vi "HOST_856.vi"() -> ()   [LabVIEW 2018]
uses:
  <vilib>/userdefined/High Color/nirio_resource_hc.ctl
  <instrlib>/niDCPower/nidcpower.llb/niDCPower Measurement Type.ctl
  <vilib>/FPGAPlugInAG/PXI-7953R/niLvFpga_Open_PXI-7953R.vi
  <vilib>/rvi/interface/common/dynamic/niFpgaDynamicAddResources.vi
  <vilib>/FPGAPlugInAG/Dynamic/niLvFpga_Reset_Dynamic.vi
  <vilib>/FPGAPlugInAG/Dynamic/niLvFpga_Run_Dynamic.vi
  <vilib>/Utility/error.llb/Error Cluster From Error Code.vi
  <vilib>/rvi/errors/niLvFpgaAdjustHostInterfaceError.vi
  <vilib>/FPGAPlugInAG/Dynamic/niLvFpga_Close_Dynamic.vi
  <vilib>/rvi/interface/nirviOpenFPGA/nirviOpenFPGA.xnode
  FPGA Bitfiles/856_FPGATarget_TARGET856_CYBaMz25M7g.lvbitx
  <vilib>/rvi/interface/nirviMethod/nirviMethod.xnode
  <vilib>/rvi/interface/nirviReadWriteControl/nirviReadWriteControl.xnode
  <vilib>/rvi/interface/nirviCloseFPGA/nirviCloseFPGA.xnode
  NiFpgaLv.dll
  <vilib>/rvi/interface/Simulation/niFpgaSimulationCallBeginRW.vi
  <vilib>/FPGAPlugInAG/Dynamic/niLvFpga_ReadFifo_Dynamic.vi
  <vilib>/rvi/errors/niLvFpgaMergeErrorWithErrorCode.vi
panel:
  in  "Tab Control":enum32{"Рабочая", "Служебная"}(tab)
  out "Image":T1(plugin-control)
  in  "Frames":path=path "D:/VPL/LabView/DOZOR_856/DOZOR_856/FRAMES"
  out "Номер образца":string="0"
  in  "LOGS":path=path "D:/VPL/LabView/DOZOR_856/DOZOR_856/LOGS"
  in  "resource name":T2="PXI1Slot6"
  in  "1":refnum<k15>="PXI1Slot3" caption="instrument handle"
  in  "0":refnum<k15>="PXI1Slot2" caption="instrument handle"
  in  "2":refnum<k15>="PXI1Slot4" caption="instrument handle"
  in  "Стоп":bool
  in  "Питание":bool
  out "PS_LOW_cur":dbl caption="measurement" format="%_6g"
  in  "PS_LOW_curlim":dbl=0.1 caption="current limit" format="%_6p"
  in  "PS_LOW, V":dbl=-8.0 caption="voltage level" format="%_6p"
  in  "-15, V":dbl=-15.0 caption="voltage level" format="%_6p"
  out "-15_cur":dbl caption="measurement" format="%_6g"
  in  "-15_curlim":dbl=0.1 caption="current limit" format="%_6p"
  out "1V_cur":dbl caption="measurement" format="%_6g"
  in  "1V_curlim":dbl=0.1 caption="current limit" format="%_6p"
  in  "1V":dbl=1.0 caption="voltage level" format="%_6p"
  in  "2V":dbl=3.100000000000001 caption="voltage level" format="%_6p"
  in  "STAB, V":dbl=10.0 caption="voltage level" format="%_6p"
  out "DD_cur":dbl caption="measurement" format="%_6g"
  out "2V_cur":dbl caption="measurement" format="%_6g"
  out "PH_LOW_cur":dbl caption="measurement" format="%_6g"
  out "RD_cur":dbl caption="measurement" format="%_6g"
  out "STAB_cur":dbl caption="measurement" format="%_6g"
  out "ADC_cur":dbl caption="measurement" format="%_6g"
  in  "DD_curlim":dbl=0.2 caption="current limit" format="%_6p"
  in  "2V_curlim":dbl=0.1 caption="current limit" format="%_6p"
  in  "PH_LOW_curlim":dbl=0.2 caption="current limit" format="%_6p"
  in  "RD_curlim":dbl=0.1 caption="current limit" format="%_6p"
  in  "STAB_curlim":dbl=0.2 caption="current limit" format="%_6p"
  in  "ADC_curlim":dbl=0.2 caption="current limit" format="%_6p"
  in  "DD, V":dbl=18.900000000000013 caption="voltage level" format="%_6p"
  in  "PH_LOW, V":dbl=-4.000000000000002 caption="voltage level" format="%_6p"
  in  "RD, V":dbl=15.099999999999996 caption="voltage level" format="%_6p"
  in  "ADC, V":dbl=6.0 caption="voltage level" format="%_6p"
  in  "Линейки":bool
  out "СКО":dbl
  in  "LED":bool
  out "Configuration":bool[](array[boolean])
  out "АЦП прошит!":bool
  in  "2/4 V":enum16{"2V", "4V"}(ring)
  in  "3CH/1CH":enum16{"3CH", "1CH"}(ring)=enum."1CH"
  in  "Какой канал?":enum16{"OUT1", "OUT2", "OUT3"}(ring)
  in  "Прошить АЦП":bool
  in  "ПРИМЕЧАНИЕ":string
  in  "Какая фотка?":string
  in  "НЕПРЕРЫВНО":bool
  in  "文韧 世男!":bool
  out "Среднее":dbl
  out "FRAME_OK":bool
  in  "Запись Кадра":bool
  out "Канал":string="1"
  in  "ПЕРЕБОР?":bool
  out "ADC":i32
  out "1V":i32
  out "2V":i32
  out "STAB":i32
  out "RD":i32
  out "DD":i32
  out "-15":i32
  out "PH":i32
  out "PS":i32
  out "ADC":bool
  out "1V":bool
  out "2V":bool
  out "STAB":bool
  out "RD":bool
  out "DD":bool
  out "-15":bool
  out "PH":bool
  out "PS":bool
  in  "SIM_SEL":bool
  out "SEL":bool
  in  "ADC_selcur":dbl=0.15 caption="current limit" format="%_6p"
  in  "STAB_selcur":dbl=0.15 caption="current limit" format="%_6p"
  in  "-15_selcur":dbl=0.01 caption="current limit" format="%_6p"
  in  "1V_selcur":dbl=0.02 caption="current limit" format="%_6p"
  in  "RD_selcur":dbl=0.01 caption="current limit" format="%_6p"
  in  "2V_curlim":dbl=0.01 caption="current limit" format="%_6p"
  in  "DD_curlim":dbl=0.1 caption="current limit" format="%_6p"
  in  "PS_LOW_curlim":dbl=0.015 caption="current limit" format="%_6p"
  in  "PH_LOW_curlim":dbl=0.12 caption="current limit" format="%_6p"
  in  "ISO":dbl=1.0
  in  "+/- OUT2":enum16{"-", "+"}(ring)=enum."+"
  in  "Смещение, до 300_OUT2":dbl
  in  "+/- OUT3":enum16{"-", "+"}(ring)=enum."+"
  in  "Смещение, до 300_OUT3":dbl
  in  "+/- OUT1":enum16{"-", "+"}(ring)=enum."+"
  in  "Смещение, до 300_OUT1":dbl
  in  "Усиление (до 6)_OUT2":u8=1
  in  "Усиление (до 6)_OUT1":u8=1
  in  "Усиление (до 6)_OUT3":u8=1
  in  "Между кадрами, мс":u8=1
  in  "Усреднение":i32=1
  out "FRAME":u16[][](array[numeric])
  out "OUT":cluster{u16, u16, u16, u16}[][](array[cluster])
  in  "HIGH":u8=18
  in  "LOW":u8=7
  in  "HOR":u16=880
  in  "RG_2":u8=5
  in  "ADC_1":u8=5
  in  "ADC_2":u8=16
  in  "CDS2_1":u8=2
  in  "CDS2_2":u8=16
  in  "CDS1_1":u8=5
  in  "CDS1_2":u8=13
  in  "PS3_2":u16=1589
  in  "PS3_1":u16=934
  in  "PS1_1":u16=715
  in  "PS1_2":u16=1809
  in  "Сколько строк?":i32=110
  in  "2017":u16=2017
  in  "PS2_1":u16=496
  in  "PS2_2":u16=1151
  in  "PS4_1":u16=277
  in  "PS4_2":u16=1371
  in  "RG_1":u8=3
  in  "PH21_2":u8=13
  in  "PH21_1":u8=3
  in  "PH11_2":u8=13
  in  "PH11_1":u8=3
  in  "10":u8=20
  # "Для обычного кабеля"
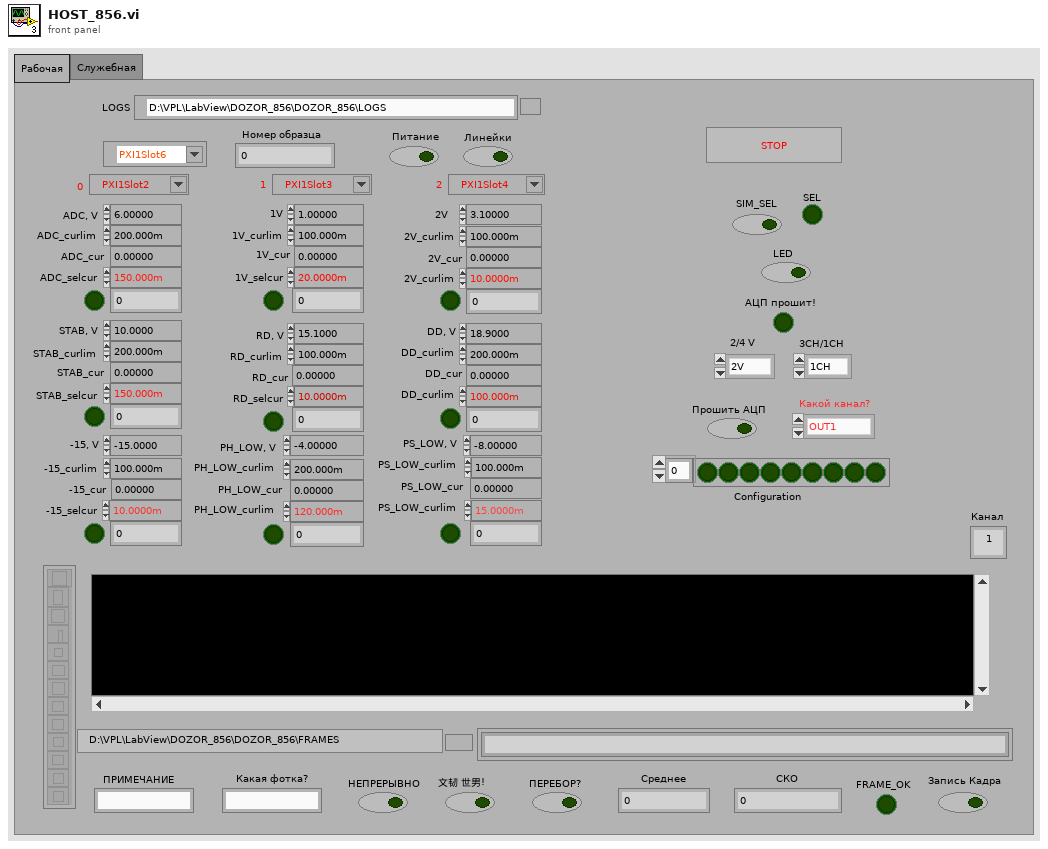
[diagram p1: front panel]
types:
  T1 = typedef "IMAQ Image.ctl" = refnum<image>
  T2 = typedef "nirio_resource_hc.ctl" = tag
  T3 = enum16{"open", "replace", "create", "open or create", "replace or create", "replace or create with confirmation"}
  T4 = typedef "niDCPower Measurement Type.ctl" = i32
  T5 = typedef "Image Type" = u32
  T6 = enum16{"Configuration", "MUX", "RED PGA", "GREEN PGA", "BLUE PGA", "RED OFF", "GREEN OFF", "BLUE OFF"}
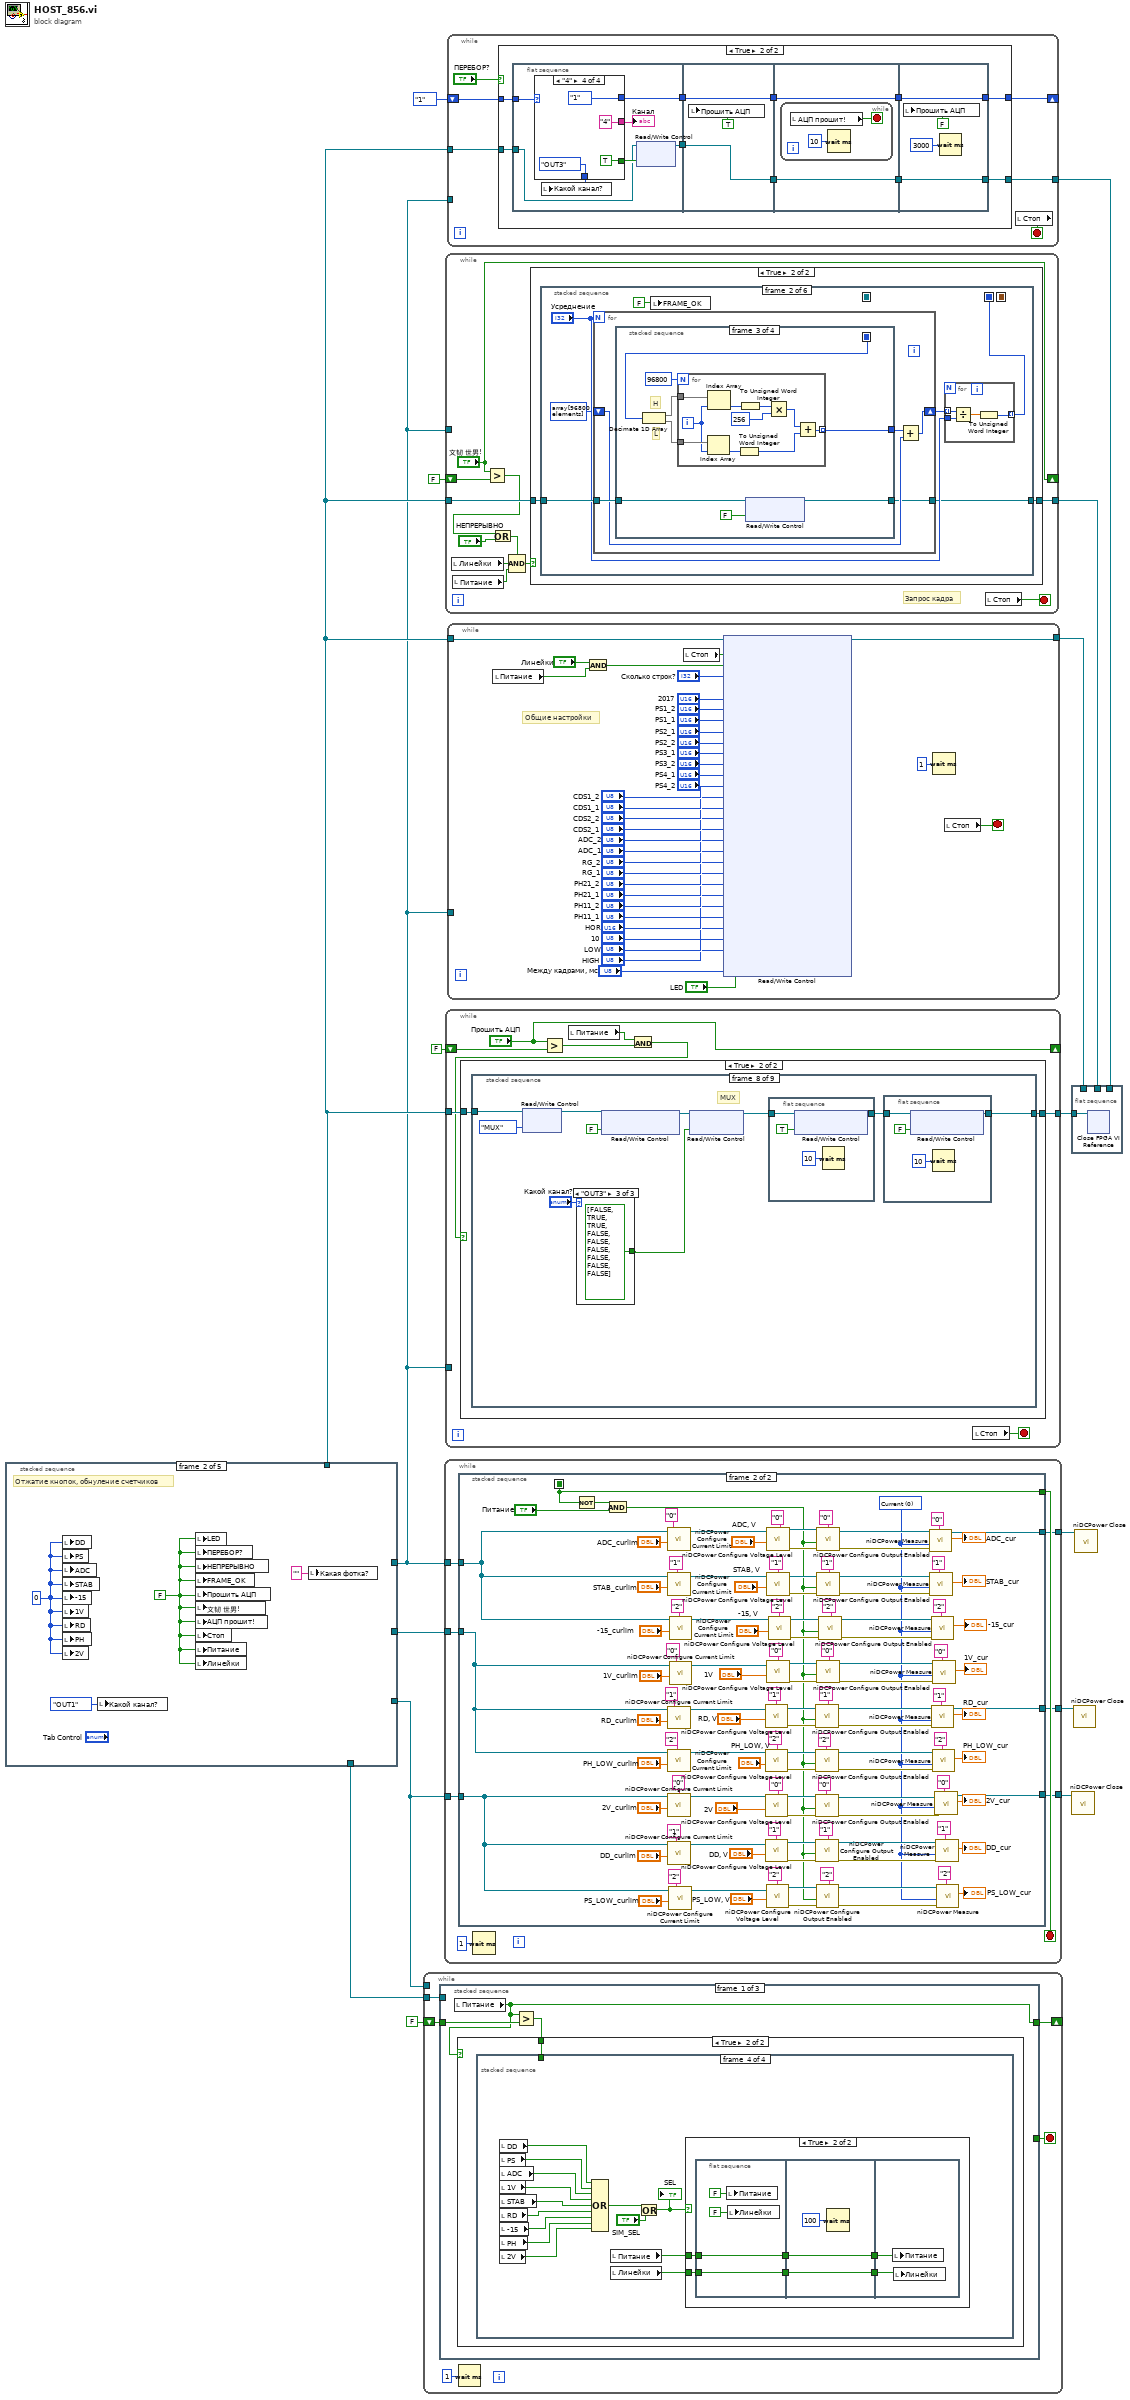
[diagram p0: block diagram]
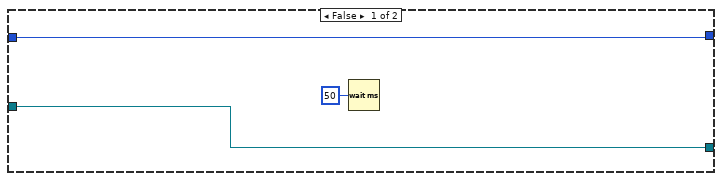
[diagram p2: hidden frame]
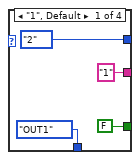
[diagram p3: hidden frame]
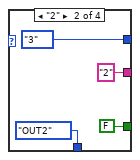
[diagram p4: hidden frame]
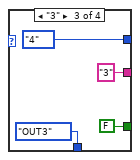
[diagram p5: hidden frame]
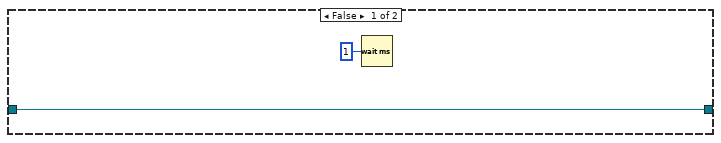
[diagram p6: hidden frame]
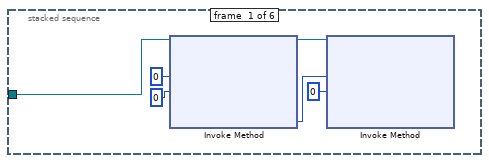
[diagram p7: hidden frame]
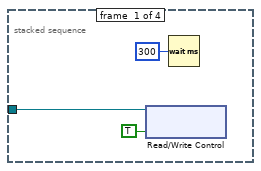
[diagram p8: hidden frame]
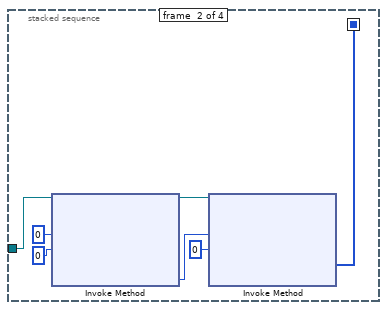
[diagram p9: hidden frame]
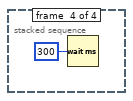
[diagram p10: hidden frame]
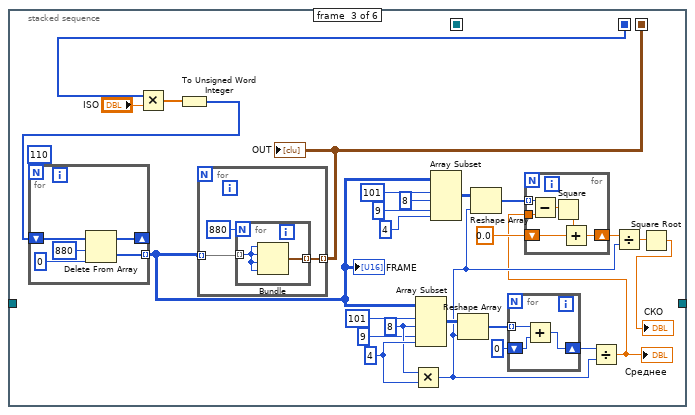
[diagram p11: hidden frame]
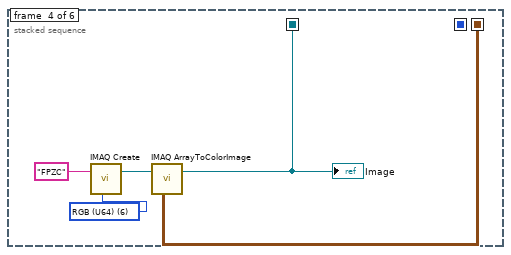
[diagram p12: hidden frame]
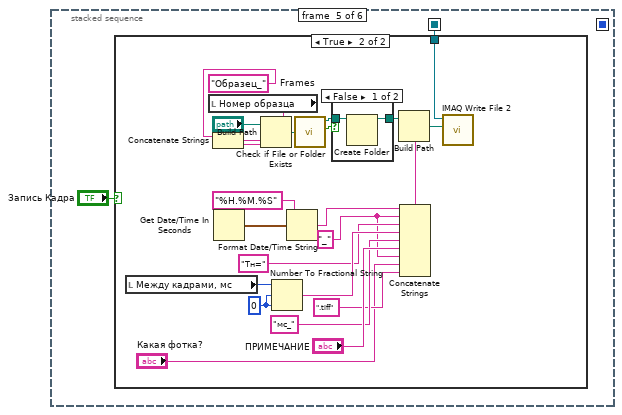
[diagram p13: hidden frame]
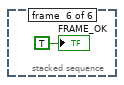
[diagram p16: hidden frame]
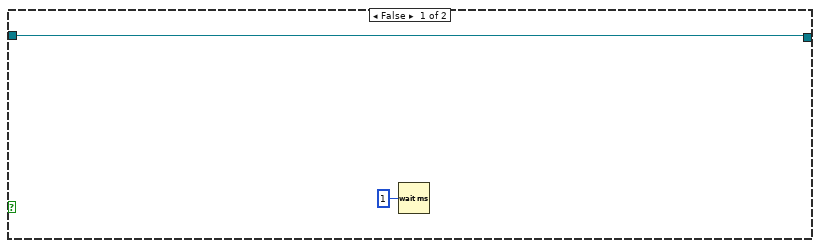
[diagram p17: hidden frame]
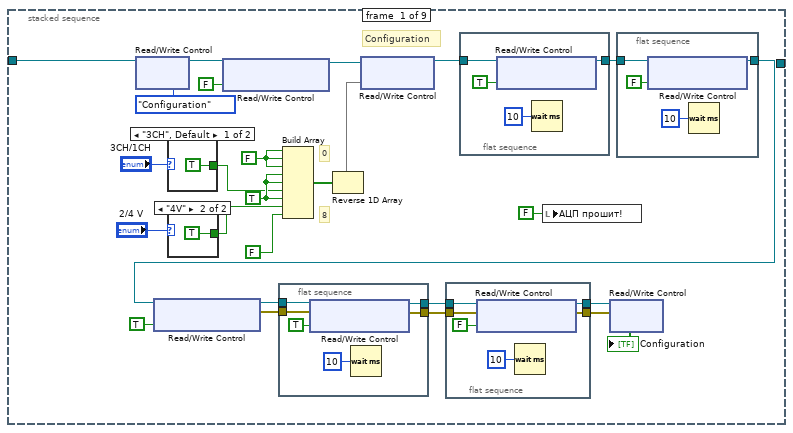
[diagram p18: hidden frame]
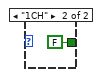
[diagram p19: hidden frame]
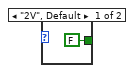
[diagram p20: hidden frame]
diagram:
  n1 = stacked-sequence {
    tunnel: [_ _ _ _ w67] -> w7
    tunnel: [_ _ _ _ w66] -> w5
    tunnel: [_ _ _ _ w65] -> w16
    tunnel: [_ _ _ w59 _] -> w9
    tunnel: [_ _ w22 _ _] -> w11
    frame #0 {
      n2 = call "Begin.vi"() -> ("Номер образца 2"=→"Номер образца":string)  [unwired: 11 in]
    }
    frame #1 {
      w18 = FALSE
      w19 = 0 ("DD")
      # "Отжатие кнопок, обнуление счетчиков"
      n3 = local write "DD"(w19) -> ()
      n4 = local write "PS"(w19) -> ()
      n5 = local write "ADC"(w19) -> ()
      n6 = local write "STAB"(w19) -> ()
      n7 = local write "-15"(w19) -> ()
      n8 = local write "1V"(w19) -> ()
      n9 = local write "RD"(w19) -> ()
      n10 = local write "PH"(w19) -> ()
      n11 = local write "2V"(w19) -> ()
      n12 = local write "Какой канал?"(enum16{"OUT1", "OUT2", "OUT3"}."OUT1" ("Какой канал?")) -> ()
      n13 = local write "LED"(w18) -> ()
      n14 = local write "ПЕРЕБОР?"(w18) -> ()
      n15 = local write "НЕПРЕРЫВНО"(w18) -> ()
      n16 = local write "FRAME_OK"(w18) -> ()
      n17 = local write "Прошить АЦП"(w18) -> ()
      n18 = local write "文韧 世男!"(w18) -> ()
      n19 = local write "АЦП прошит!"(w18) -> ()
      n20 = local write "Стоп"(w18) -> ()
      n21 = local write "Питание"(w18) -> ()
      n22 = local write "Линейки"(w18) -> ()
      n23 = local write "Какая фотка?"("" ("Какая фотка?")) -> ()
    }
    frame #2 {
      w24 = "\t"
      n24 = local read "Номер образца"() -> (w51:string)
      n25 = Build Path(base path="LOGS", name or relative path=w51) -> (appended path=w48:path)
      n26 = Get Date/Time In Seconds() -> (seconds since 1Jan1904=w45:timestamp)
      n27 = call <vilib>:"Check if File or Folder Exists.vi"("path"=w48) -> ("file or folder exists?"=w49:bool, "dup path"=w50:path)  [unwired: 8 in, 1 out]
      n28 = Format Date/Time String(time format string (%c)="%d %H.%M.%S", seconds (now)=w45) -> (date/time string=w43:string)  [unwired: 1 in]
      n29 = case shown="False" w49 {
        tunnel: w50 -> [w57 w58]
        tunnel: [w56 w58] -> w40
        frame False {
          n30 = Create Folder(path (use dialog)=w57) -> (created path=w56:path)  [unwired: 2 in, 2 out]
        }
        frame True {
        }
      }
      n31 = Concatenate Strings(w43, ".xls" ("string")) -> (w42:string)
      n32 = Build Path(base path=w40, name or relative path=w42) -> (appended path=w44:path)
      n33 = Open/Create/Replace File(file path (use dialog)=w44, operation (0:open)=T3."open or create", access (0:read/write)=enum16{"read/write", "read-only", "write-only"}."read/write") -> (refnum out=w46:refnum<file>)  [unwired: 3 in, 2 out]
      n34 = case shown="True" TRUE {
        tunnel: w46 -> [w52 w55]
        tunnel: [w52 w53] -> w41
        frame False {
        }
        frame True {
          n35 = Set File Position(refnum=w55, from (0:start)=enum16{"start", "end", "current"}."end") -> (refnum out=w53:refnum<file>)  [unwired: 2 in, 1 out]
        }
      }
      n36 = Format Into String(initial string=w41, "Time" ("input 1"), w24, "ADC_cur", w24, "STAB_cur", w24, "-15_cur", w24, "1_cur", w24, "RD_cur", w24, "PH_LOW_cur", w24, "2V_cur", w24, "DD_cur", w24, "PS_LOW_cur", "\r\n") -> (resulting string=w22:refnum<file>)  [unwired: 2 in, 1 out]
    }
    frame #3 {
      n37 = xnode "Open FPGA VI Reference"("resource name"="resource name") -> ("FPGA VI Reference Out"=w60:refnum<k20>, "error out"=w62:errorcluster)  [unwired: 1 in]
      n38 = xnode "Invoke Method"("FPGA VI Reference In"=w60, "error in"=w62) -> ("FPGA VI Reference Out"=w63:refnum<k20>, "error out"=w61:errorcluster)
      n39 = xnode "Invoke Method"("FPGA VI Reference In"=w63, "error in"=w61) -> ("FPGA VI Reference Out"=w59:refnum<k20>)  [unwired: 1 in, 1 out]
    }
    frame #4 {
      n40 = call <instrlib>:"niDCPower Initialize.vi"("resource name"="2") -> ("error out"=w73:errorcluster, "instrument handle out"=w70:refnum<k15>)  [unwired: 3 in, 6 out]
      n41 = call <instrlib>:"niDCPower Initialize.vi"("resource name"="1") -> ("error out"=w71:errorcluster, "instrument handle out"=w68:refnum<k15>)  [unwired: 3 in, 6 out]
      n42 = call <instrlib>:"niDCPower Initialize.vi"("resource name"="0") -> ("error out"=w72:errorcluster, "instrument handle out"=w69:refnum<k15>)  [unwired: 3 in, 6 out]
      n43 = call <instrlib>:"niDCPower Configure Voltage Level.vi"("error in (no error)"=w73, "voltage level"=0.0, "channel name"="0,1,2", "instrument handle"=w70) -> ("instrument handle out"=w67:refnum<k15>)  [unwired: 6 in, 1 out]
      n44 = call <instrlib>:"niDCPower Configure Voltage Level.vi"("error in (no error)"=w71, "voltage level"=0.0, "channel name"="0,1,2", "instrument handle"=w68) -> ("instrument handle out"=w65:refnum<k15>)  [unwired: 6 in, 1 out]
      n45 = call <instrlib>:"niDCPower Configure Voltage Level.vi"("error in (no error)"=w72, "voltage level"=0.0, "channel name"="0,1,2", "instrument handle"=w69) -> ("instrument handle out"=w66:refnum<k15>)  [unwired: 6 in, 1 out]
    }
  }
  n46 = while {
    shift-right: [w85] -> _
    shift-left: FALSE ("Питание") -> [w86]
    tunnel: w11 -> [w83]
    tunnel: w7 -> [_]
    stop <- w84 stop-if-true
    n47 = stacked-sequence {
      tunnel: [_ _ w228] -> w84
      tunnel: w86 -> [w90 _ _]
      tunnel: [w89 _ _] -> w85
      tunnel: w83 -> [_ w193 _]
      frame #0 {
        n48 = local read "Питание"() -> (w89:bool)
        n49 = Greater?(x=w89, y=w90) -> (0:w88:bool)
        n50 = case shown="True" w89 {
          tunnel: w88 -> [_ w91]
          frame False {
          }
          frame True {
            n51 = stacked-sequence {
              tunnel: w91 -> [w92 _ _ _]
              frame #0 {
                n52 = local read "SEL"() -> (w93:bool)
                n53 = Or(x=w92, y=w93) -> (x .or. y?=w94:bool)
                n54 = case shown="True" w94 {
                  frame False {
                  }
                  frame True {
                    n55 = flat-sequence {
                      frame #0 {
                        n56 = Wait (ms)(milliseconds to wait=u32 500) -> ()  [unwired: 1 out]
                      }
                      frame #1 {
                        n57 = local write "Прошить АЦП"(TRUE ("Прошить АЦП")) -> ()
                        n58 = Wait (ms)(milliseconds to wait=u32 100) -> ()  [unwired: 1 out]
                      }
                      frame #2 {
                        n59 = local write "Прошить АЦП"(FALSE ("Прошить АЦП")) -> ()
                      }
                    }
                  }
                }
              }
              frame #1 {
                n60 = local read "STAB_cur"() -> (w121:dbl)
                n61 = local read "1V_cur"() -> (w119:dbl)
                n62 = local read "2V_cur"() -> (w116:dbl)
                n63 = local read "ADC_cur"() -> (w124:dbl)
                n64 = Greater?(x=w119, y="1V_selcur") -> (0:→"1V":bool)
                n65 = Greater?(x=w116, y="2V_curlim") -> (0:→"2V":bool)
                n66 = Greater?(x=w121, y="STAB_selcur") -> (0:→"STAB":bool)
                n67 = Greater?(x=w124, y="ADC_selcur") -> (0:→"ADC":bool)
                n68 = local read "PH_LOW_cur"() -> (w104:dbl)
                n69 = local read "PS_LOW_cur"() -> (w113:dbl)
                n70 = local read "DD_cur"() -> (w110:dbl)
                n71 = local read "-15_cur"() -> (w101:dbl)
                n72 = local read "RD_cur"() -> (w107:dbl)
                n73 = Greater?(x=w107, y="RD_selcur") -> (0:→"RD":bool)
                n74 = Greater?(x=w104, y="PH_LOW_curlim") -> (0:→"PH":bool)
                n75 = Greater?(x=w101, y="-15_selcur") -> (0:→"-15":bool)
                n76 = Greater?(x=w110, y="DD_curlim") -> (0:→"DD":bool)
                n77 = Greater?(x=w113, y="PS_LOW_curlim") -> (0:→"PS":bool)
              }
              frame #2 {
                n78 = local read "ADC"() -> (w132:bool)
                n79 = local read "STAB"() -> (w131:bool)
                n80 = local read "-15"() -> (w130:bool)
                n81 = local read "1V"() -> (w129:bool)
                n82 = local read "DD"() -> (w134:bool)
                n83 = local read "PS"() -> (w133:bool)
                n84 = case shown="True" w134 {
                  frame False {
                  }
                  frame True {
                    n85 = local read "DD"() -> (w152:i32)
                    n86 = Increment(x=w152) -> (x+1=→"DD":i32)
                  }
                }
                n87 = case shown="True" w133 {
                  frame False {
                  }
                  frame True {
                    n88 = local read "PS"() -> (w150:i32)
                    n89 = Increment(x=w150) -> (x+1=→"PS":i32)
                  }
                }
                n90 = case shown="True" w132 {
                  frame False {
                  }
                  frame True {
                    n91 = local read "ADC"() -> (w148:i32)
                    n92 = Increment(x=w148) -> (x+1=→"ADC":i32)
                  }
                }
                n93 = case shown="True" w131 {
                  frame False {
                  }
                  frame True {
                    n94 = local read "STAB"() -> (w146:i32)
                    n95 = Increment(x=w146) -> (x+1=→"STAB":i32)
                  }
                }
                n96 = case shown="True" w130 {
                  frame False {
                  }
                  frame True {
                    n97 = local read "-15"() -> (w144:i32)
                    n98 = Increment(x=w144) -> (x+1=→"-15":i32)
                  }
                }
                n99 = case shown="True" w129 {
                  frame False {
                  }
                  frame True {
                    n100 = local read "1V"() -> (w142:i32)
                    n101 = Increment(x=w142) -> (x+1=→"1V":i32)
                  }
                }
                n102 = local read "RD"() -> (w128:bool)
                n103 = local read "2V"() -> (w126:bool)
                n104 = local read "PH"() -> (w127:bool)
                n105 = case shown="True" w127 {
                  frame False {
                  }
                  frame True {
                    n106 = local read "PH"() -> (w138:i32)
                    n107 = Increment(x=w138) -> (x+1=→"PH":i32)
                  }
                }
                n108 = case shown="True" w128 {
                  frame False {
                  }
                  frame True {
                    n109 = local read "RD"() -> (w140:i32)
                    n110 = Increment(x=w140) -> (x+1=→"RD":i32)
                  }
                }
                n111 = case shown="True" w126 {
                  frame False {
                  }
                  frame True {
                    n112 = local read "2V"() -> (w136:i32)
                    n113 = Increment(x=w136) -> (x+1=→"2V":i32)
                  }
                }
              }
              frame #3 {
                n114 = local read "DD"() -> (w165:bool)
                n115 = local read "PS"() -> (w164:bool)
                n116 = local read "ADC"() -> (w163:bool)
                n117 = local read "1V"() -> (w162:bool)
                n118 = local read "STAB"() -> (w161:bool)
                n119 = local read "RD"() -> (w160:bool)
                n120 = local read "-15"() -> (w159:bool)
                n121 = local read "PH"() -> (w158:bool)
                n122 = local read "2V"() -> (w157:bool)
                n123 = Compound Arithmetic op=OR(w165, w164, w163, w162, w161, w160, w159, w158, w157) -> (w156:bool)
                n124 = local read "Питание"() -> (w155:bool)
                n125 = local read "Линейки"() -> (w154:bool)
                n126 = Or(x=w156, y="SIM_SEL") -> (x .or. y?=w153:bool)
                "SEL" <- w153
                n127 = case shown="True" w153 {
                  tunnel: w155 -> [_ w173]
                  tunnel: w154 -> [_ w172]
                  frame False {
                    n128 = Wait (ms)(milliseconds to wait=u32 1) -> ()  [unwired: 1 out]
                  }
                  frame True {
                    n129 = flat-sequence {
                      tunnel: w173 -> [w177]
                      tunnel: w172 -> [w176]
                      tunnel: [w177] -> w170
                      tunnel: [w176] -> w168
                      tunnel: [w179] -> w171
                      tunnel: w170 -> [w179]
                      tunnel: [w178] -> w169
                      tunnel: w168 -> [w178]
                      tunnel: w171 -> [w182]
                      tunnel: w169 -> [w181]
                      frame #0 {
                        n130 = local write "Питание"(FALSE ("Питание")) -> ()
                        n131 = local write "Линейки"(FALSE ("Линейки")) -> ()
                      }
                      frame #1 {
                        n132 = Wait (ms)(milliseconds to wait=u32 100) -> ()  [unwired: 1 out]
                      }
                      frame #2 {
                        n133 = local write "Питание"(w182) -> ()
                        n134 = local write "Линейки"(w181) -> ()
                      }
                    }
                  }
                }
              }
            }
          }
        }
      }
      frame #1 {
        w203 = i16 0 ("width (-)")
        w206 = i16 3 ("width (-)")
        w204 = "\t"
        # "Логирование данных"
        n135 = local read "STAB"() -> (w201:i32)
        n136 = local read "ADC"() -> (w202:i32)
        n137 = local read "-15"() -> (w200:i32)
        n138 = local read "PH"() -> (w197:i32)
        n139 = local read "DD"() -> (w195:i32)
        n140 = local read "RD"() -> (w198:i32)
        n141 = local read "1V"() -> (w199:i32)
        n142 = local read "2V"() -> (w196:i32)
        n143 = local read "PS"() -> (w194:i32)
        n144 = Number To Fractional String(number=w202, width (-)=w203, precision (6)=w203) -> (F-format string=w191:string)  [unwired: 1 in]
        n145 = Number To Fractional String(number=w201, width (-)=w203, precision (6)=w203) -> (F-format string=w190:string)  [unwired: 1 in]
        n146 = Number To Fractional String(number=w200, width (-)=w203, precision (6)=w203) -> (F-format string=w189:string)  [unwired: 1 in]
        n147 = Number To Fractional String(number=w199, width (-)=w203, precision (6)=w203) -> (F-format string=w188:string)  [unwired: 1 in]
        n148 = Number To Fractional String(number=w198, width (-)=w203, precision (6)=w203) -> (F-format string=w187:string)  [unwired: 1 in]
        n149 = Number To Fractional String(number=w197, width (-)=w203, precision (6)=w203) -> (F-format string=w186:string)  [unwired: 1 in]
        n150 = Number To Fractional String(number=w196, width (-)=w203, precision (6)=w203) -> (F-format string=w185:string)  [unwired: 1 in]
        n151 = Number To Fractional String(number=w195, width (-)=w203, precision (6)=w203) -> (F-format string=w184:string)  [unwired: 1 in]
        n152 = Number To Fractional String(number=w194, width (-)=w203, precision (6)=w203) -> (F-format string=w183:string)  [unwired: 1 in]
        n153 = local read "PH_LOW_cur"() -> (w210:dbl)
        n154 = local read "PS_LOW_cur"() -> (w207:dbl)
        n155 = local read "STAB_cur"() -> (w214:dbl)
        n156 = local read "ADC_cur"() -> (w215:dbl)
        n157 = local read "DD_cur"() -> (w208:dbl)
        n158 = local read "-15_cur"() -> (w213:dbl)
        n159 = local read "RD_cur"() -> (w211:dbl)
        n160 = local read "1V_cur"() -> (w212:dbl)
        n161 = local read "2V_cur"() -> (w209:dbl)
        n162 = Number To Fractional String(number=w215, width (-)=w206, precision (6)=w206) -> (F-format string=w224:string)  [unwired: 1 in]
        n163 = Number To Fractional String(number=w214, width (-)=w206, precision (6)=w206) -> (F-format string=w223:string)  [unwired: 1 in]
        n164 = Number To Fractional String(number=w213, width (-)=w206, precision (6)=w206) -> (F-format string=w222:string)  [unwired: 1 in]
        n165 = Number To Fractional String(number=w212, width (-)=w206, precision (6)=w206) -> (F-format string=w221:string)  [unwired: 1 in]
        n166 = Number To Fractional String(number=w211, width (-)=w206, precision (6)=w206) -> (F-format string=w220:string)  [unwired: 1 in]
        n167 = Number To Fractional String(number=w210, width (-)=w206, precision (6)=w206) -> (F-format string=w219:string)  [unwired: 1 in]
        n168 = Number To Fractional String(number=w209, width (-)=w206, precision (6)=w206) -> (F-format string=w218:string)  [unwired: 1 in]
        n169 = Number To Fractional String(number=w208, width (-)=w206, precision (6)=w206) -> (F-format string=w217:string)  [unwired: 1 in]
        n170 = Number To Fractional String(number=w207, width (-)=w206, precision (6)=w206) -> (F-format string=w216:string)  [unwired: 1 in]
        n171 = Get Date/Time In Seconds() -> (seconds since 1Jan1904=w227:timestamp)
        n172 = Format Date/Time String(time format string (%c)="%d %H:%M:%S:%3u", seconds (now)=w227) -> (date/time string=w225:string)  [unwired: 1 in]
        n173 = Concatenate Strings(w225, w204, w224, w204, w223, w204, w222, w204, w221, w204, w220, w204, w219, w204, w218, w204, w217, w204, w216, w204, w191, w204, w190, w204, w189, w204, w188, w204, w187, w204, w186, w204, w185, w204, w184, w204, w183, "\r\n") -> (w226:string)
        n174 = Format Into String(initial string=w193, w226) -> ()  [unwired: 2 in, 2 out]
      }
      frame #2 {
        n175 = local read "Стоп"() -> (w228:bool)
      }
    }
    n176 = Wait (ms)(milliseconds to wait=u32 1) -> ()  [unwired: 1 out]
  }
  n177 = while {
    tunnel: w5 -> [w235]
    tunnel: w16 -> [w234]
    tunnel: w7 -> [w233]
    tunnel: [w231] -> w15
    tunnel: [w230] -> w14
    tunnel: [w229] -> w13
    stop <- w232 stop-if-true
    n178 = stacked-sequence {
      seq-local: ["Стоп" _] -> [_ w238]
      tunnel: w233 -> [_ w243]
      tunnel: [_ w284] -> w231
      tunnel: [_ w283] -> w230
      tunnel: [_ w282] -> w229
      tunnel: w235 -> [_ w242]
      tunnel: w234 -> [_ w241]
      tunnel: [_ w238] -> w232
      frame #0 {
      }
      frame #1 {
        w244 = T4 0 items=["Current", "Voltage"] ("measurement type")
        n179 = Not(x=w238) -> (.not. x?=w257:bool)
        n180 = And(x=w257, y="Питание") -> (x .and. y?=w239:bool)
        n181 = call <instrlib>:"niDCPower Configure Current Limit.vi"("current limit"="ADC_curlim", "channel name"="0", "instrument handle"=w242) -> ("instrument handle out"=w319:refnum<k15>)  [unwired: 7 in, 1 out]
        n182 = call <instrlib>:"niDCPower Configure Current Limit.vi"("current limit"="STAB_curlim", "channel name"="1", "instrument handle"=w242) -> ("instrument handle out"=w320:refnum<k15>)  [unwired: 7 in, 1 out]
        n183 = call <instrlib>:"niDCPower Configure Current Limit.vi"("current limit"="RD_curlim", "channel name"="1", "instrument handle"=w241) -> ("instrument handle out"=w321:refnum<k15>)  [unwired: 7 in, 1 out]
        n184 = call <instrlib>:"niDCPower Configure Current Limit.vi"("current limit"="PH_LOW_curlim", "channel name"="2", "instrument handle"=w241) -> ("instrument handle out"=w322:refnum<k15>)  [unwired: 7 in, 1 out]
        n185 = call <instrlib>:"niDCPower Configure Current Limit.vi"("current limit"="2V_curlim", "channel name"="0", "instrument handle"=w243) -> ("instrument handle out"=w323:refnum<k15>)  [unwired: 7 in, 1 out]
        n186 = call <instrlib>:"niDCPower Configure Current Limit.vi"("current limit"="DD_curlim", "channel name"="1", "instrument handle"=w243) -> ("instrument handle out"=w324:refnum<k15>)  [unwired: 7 in, 1 out]
        n187 = call <instrlib>:"niDCPower Configure Current Limit.vi"("current limit"="PS_LOW_curlim", "channel name"="2", "instrument handle"=w243) -> ("instrument handle out"=w250:refnum<k15>)  [unwired: 7 in, 1 out]
        n188 = call <instrlib>:"niDCPower Configure Current Limit.vi"("current limit"="-15_curlim", "channel name"="2", "instrument handle"=w242) -> ("instrument handle out"=w264:refnum<k15>)  [unwired: 7 in, 1 out]
        n189 = call <instrlib>:"niDCPower Configure Current Limit.vi"("current limit"="1V_curlim", "channel name"="0", "instrument handle"=w241) -> ("instrument handle out"=w275:refnum<k15>)  [unwired: 7 in, 1 out]
        n190 = call <instrlib>:"niDCPower Configure Voltage Level.vi"("voltage level"="RD, V", "channel name"="1", "instrument handle"=w321) -> ("error out"=w302:errorcluster, "instrument handle out"=w299:refnum<k15>)  [unwired: 7 in]
        n191 = call <instrlib>:"niDCPower Configure Voltage Level.vi"("voltage level"="PH_LOW, V", "channel name"="2", "instrument handle"=w322) -> ("error out"=w301:errorcluster, "instrument handle out"=w300:refnum<k15>)  [unwired: 7 in]
        n192 = call <instrlib>:"niDCPower Configure Voltage Level.vi"("voltage level"="2V", "channel name"="0", "instrument handle"=w323) -> ("error out"=w311:errorcluster, "instrument handle out"=w314:refnum<k15>)  [unwired: 7 in]
        n193 = call <instrlib>:"niDCPower Configure Voltage Level.vi"("voltage level"="DD, V", "channel name"="1", "instrument handle"=w324) -> ("error out"=w312:errorcluster, "instrument handle out"=w313:refnum<k15>)  [unwired: 7 in]
        n194 = call <instrlib>:"niDCPower Configure Voltage Level.vi"("voltage level"="PS_LOW, V", "channel name"="2", "instrument handle"=w250) -> ("error out"=w253:errorcluster, "instrument handle out"=w252:refnum<k15>)  [unwired: 7 in]
        n195 = call <instrlib>:"niDCPower Configure Voltage Level.vi"("voltage level"="ADC, V", "channel name"="0", "instrument handle"=w319) -> ("error out"=w289:errorcluster, "instrument handle out"=w292:refnum<k15>)  [unwired: 7 in]
        n196 = call <instrlib>:"niDCPower Configure Voltage Level.vi"("voltage level"="STAB, V", "channel name"="1", "instrument handle"=w320) -> ("error out"=w290:errorcluster, "instrument handle out"=w291:refnum<k15>)  [unwired: 7 in]
        n197 = call <instrlib>:"niDCPower Configure Voltage Level.vi"("voltage level"="1V", "channel name"="0", "instrument handle"=w275) -> ("error out"=w279:errorcluster, "instrument handle out"=w280:refnum<k15>)  [unwired: 7 in]
        n198 = call <instrlib>:"niDCPower Configure Voltage Level.vi"("voltage level"="-15, V", "channel name"="2", "instrument handle"=w264) -> ("error out"=w267:errorcluster, "instrument handle out"=w266:refnum<k15>)  [unwired: 7 in]
        n199 = call <instrlib>:"niDCPower Configure Output Enabled.vi"("error in (no error)"=w302, "output enabled"=w239, "channel name"="1", "instrument handle"=w299) -> ("error out"=w348:errorcluster, "instrument handle out"=w341:refnum<k15>)  [unwired: 6 in]
        n200 = call <instrlib>:"niDCPower Configure Output Enabled.vi"("error in (no error)"=w301, "output enabled"=w239, "channel name"="2", "instrument handle"=w300) -> ("error out"=w343:errorcluster, "instrument handle out"=w342:refnum<k15>)  [unwired: 6 in]
        n201 = call <instrlib>:"niDCPower Configure Output Enabled.vi"("error in (no error)"=w311, "output enabled"=w239, "channel name"="0", "instrument handle"=w314) -> ("error out"=w345:errorcluster, "instrument handle out"=w344:refnum<k15>)  [unwired: 6 in]
        n202 = call <instrlib>:"niDCPower Configure Output Enabled.vi"("error in (no error)"=w312, "output enabled"=w239, "channel name"="1", "instrument handle"=w313) -> ("error out"=w346:errorcluster, "instrument handle out"=w347:refnum<k15>)  [unwired: 6 in]
        n203 = call <instrlib>:"niDCPower Configure Output Enabled.vi"("error in (no error)"=w253, "output enabled"=w239, "channel name"="2", "instrument handle"=w252) -> ("error out"=w247:errorcluster, "instrument handle out"=w246:refnum<k15>)  [unwired: 6 in]
        n204 = call <instrlib>:"niDCPower Configure Output Enabled.vi"("error in (no error)"=w289, "output enabled"=w239, "channel name"="0", "instrument handle"=w292) -> ("error out"=w332:errorcluster, "instrument handle out"=w331:refnum<k15>)  [unwired: 6 in]
        n205 = call <instrlib>:"niDCPower Configure Output Enabled.vi"("error in (no error)"=w290, "output enabled"=w239, "channel name"="1", "instrument handle"=w291) -> ("error out"=w333:errorcluster, "instrument handle out"=w334:refnum<k15>)  [unwired: 6 in]
        n206 = call <instrlib>:"niDCPower Configure Output Enabled.vi"("error in (no error)"=w279, "output enabled"=w239, "channel name"="0", "instrument handle"=w280) -> ("error out"=w271:errorcluster, "instrument handle out"=w272:refnum<k15>)  [unwired: 6 in]
        n207 = call <instrlib>:"niDCPower Configure Output Enabled.vi"("error in (no error)"=w267, "output enabled"=w239, "channel name"="2", "instrument handle"=w266) -> ("error out"=w262:errorcluster, "instrument handle out"=w261:refnum<k15>)  [unwired: 6 in]
        n208 = call <instrlib>:"niDCPower Measure.vi"("error in (no error)"=w332, "measurement type"=w244, "channel name"="0", "instrument handle"=w331) -> ("measurement"=→"ADC_cur":dbl, "instrument handle out"=w284:refnum<k15>)  [unwired: 5 in, 1 out]
        n209 = call <instrlib>:"niDCPower Measure.vi"("error in (no error)"=w333, "measurement type"=w244, "channel name"="1", "instrument handle"=w334) -> ("measurement"=→"STAB_cur":dbl)  [unwired: 5 in, 2 out]
        n210 = call <instrlib>:"niDCPower Measure.vi"("error in (no error)"=w262, "measurement type"=w244, "channel name"="2", "instrument handle"=w261) -> ("measurement"=→"-15_cur":dbl)  [unwired: 5 in, 2 out]
        n211 = call <instrlib>:"niDCPower Measure.vi"("error in (no error)"=w348, "measurement type"=w244, "channel name"="1", "instrument handle"=w341) -> ("measurement"=→"RD_cur":dbl, "instrument handle out"=w283:refnum<k15>)  [unwired: 5 in, 1 out]
        n212 = call <instrlib>:"niDCPower Measure.vi"("error in (no error)"=w343, "measurement type"=w244, "channel name"="2", "instrument handle"=w342) -> ("measurement"=→"PH_LOW_cur":dbl)  [unwired: 5 in, 2 out]
        n213 = call <instrlib>:"niDCPower Measure.vi"("error in (no error)"=w271, "measurement type"=w244, "channel name"="0", "instrument handle"=w272) -> ("measurement"=→"1V_cur":dbl)  [unwired: 5 in, 2 out]
        n214 = call <instrlib>:"niDCPower Measure.vi"("error in (no error)"=w345, "measurement type"=w244, "channel name"="0", "instrument handle"=w344) -> ("measurement"=→"2V_cur":dbl, "instrument handle out"=w282:refnum<k15>)  [unwired: 5 in, 1 out]
        n215 = call <instrlib>:"niDCPower Measure.vi"("error in (no error)"=w346, "measurement type"=w244, "channel name"="1", "instrument handle"=w347) -> ("measurement"=→"DD_cur":dbl)  [unwired: 5 in, 2 out]
        n216 = call <instrlib>:"niDCPower Measure.vi"("error in (no error)"=w247, "measurement type"=w244, "channel name"="2", "instrument handle"=w246) -> ("measurement"=→"PS_LOW_cur":dbl)  [unwired: 5 in, 2 out]
      }
    }
    n217 = Wait (ms)(milliseconds to wait=u32 1) -> ()  [unwired: 1 out]
  }
  n218 = while {
    tunnel: w9 -> [w366]
    shift-right: ["文韧 世男!"] -> _
    shift-left: FALSE ("文韧 世男!") -> [w362]
    tunnel: [w357] -> w2
    tunnel: w5 -> [_]
    stop <- w367 stop-if-true
    # "Запрос кадра"
    n219 = local read "Линейки"() -> (w365:bool)
    n220 = local read "Питание"() -> (w364:bool)
    n221 = Greater?(x="文韧 世男!", y=w362) -> (0:w359:bool)
    n222 = Or(x=w359, y="НЕПРЕРЫВНО") -> (x .or. y?=w360:bool)
    n223 = Compound Arithmetic op=AND(w360, w365, w364) -> (w363:bool)
    n224 = case shown="True" w363 {
      tunnel: w366 -> [w368 w371]
      tunnel: [w368 w370] -> w357
      frame False {
        n225 = Wait (ms)(milliseconds to wait=u32 1) -> ()  [unwired: 1 out]
      }
      frame True {
        n226 = stacked-sequence {
          seq-local: [_ w383 _ _ _ _] -> [_ _ w438 _ _ _]
          seq-local: [_ _ w448 _ _ _] -> [_ _ _ w470 _ _]
          seq-local: [_ _ _ w469 _ _] -> [_ _ _ _ w474 _]
          tunnel: w371 -> [w372 w384 _ _ _ _]
          tunnel: [_ w378 _ _ _ _] -> w370
          frame #0 {
            n227 = xnode "Invoke Method"("FPGA VI Reference In"=w372, "Number of Elements"=u32 0, "Timeout (ms)"=0) -> ("FPGA VI Reference Out"=w377:refnum<k20>, "Elements Remaining"=w376:u32)  [unwired: 1 in, 2 out]
            n228 = xnode "Invoke Method"("FPGA VI Reference In"=w377, "Number of Elements"=w376, "Timeout (ms)"=0) -> ()  [unwired: 1 in, 4 out]
          }
          frame #1 {
            n229 = for {
              N: "Усреднение" -> [_]
              tunnel: w384 -> [w393]
              shift-right: [w390] -> w382
              shift-left: u64[] array[96800 elements] -> [w391]
              tunnel: [w389] -> w378
              n230 = stacked-sequence {
                seq-local: [_ w398 _ _] -> [_ _ w411 _]
                tunnel: w393 -> [w395 w397 w405 _]
                tunnel: [_ _ w407 _] -> w392
                tunnel: [_ _ w404 _] -> w389
                frame #0 {
                  n231 = xnode "Read/Write Control"("FPGA VI Reference In"=w395, "Кадр в FIFO"=TRUE) -> ()  [unwired: 1 in, 2 out]
                  n232 = Wait (ms)(milliseconds to wait=u32 300) -> ()  [unwired: 1 out]
                }
                frame #1 {
                  n233 = xnode "Invoke Method"("FPGA VI Reference In"=w397, "Number of Elements"=u32 0, "Timeout (ms)"=0) -> ("FPGA VI Reference Out"=w400:refnum<k20>, "Elements Remaining"=w399:u32)  [unwired: 1 in, 2 out]
                  n234 = xnode "Invoke Method"("FPGA VI Reference In"=w400, "Number of Elements"=w399, "Timeout (ms)"=0) -> ("Data"=w398:u8[])  [unwired: 1 in, 3 out]
                }
                frame #2 {
                  # "L"
                  # "H"
                  n235 = Decimate 1D Array(w411) -> (w410:u8[], w409:u8[])
                  n236 = for {
                    N: 96800 -> [_]
                    tunnel: w410 -> [w421]
                    tunnel: w409 -> [w420]
                    tunnel: [w412] -> w407 mode=indexing
                    i -> [w419]
                    n237 = Index Array(array=w420, index=w419) -> (element=w417:u8)
                    n238 = Index Array(array=w421, index=w419) -> (element=w418:u8)
                    n239 = To Unsigned Word Integer(number=w417) -> (unsigned 16bit integer=w413:u16)
                    n240 = To Unsigned Word Integer(number=w418) -> (unsigned 16bit integer=w416:u16)
                    n241 = Multiply(x=w416, y=u16 256) -> (x*y=w414:u16)
                    n242 = Add(x=w414, y=w413) -> (x+y=w412:u16)
                  }
                  n243 = xnode "Read/Write Control"("FPGA VI Reference In"=w405, "Кадр в FIFO"=FALSE) -> ("FPGA VI Reference Out"=w404:refnum<k20>)  [unwired: 1 in, 1 out]
                }
                frame #3 {
                  n244 = Wait (ms)(milliseconds to wait=u32 300) -> ()  [unwired: 1 out]
                }
              }
              n245 = Add(x=w392, y=w391) -> (x+y=w390:u64[])
            }
            n246 = local write "FRAME_OK"(FALSE ("FRAME_OK")) -> ()
            n247 = for {
              tunnel: w382 -> [w388] mode=indexing
              tunnel: "Усреднение" -> [w387]
              tunnel: [w385] -> w383 mode=indexing
              n248 = Divide(x=w388, y=w387) -> (x/y=w386:dbl)
              n249 = To Unsigned Word Integer(number=w386) -> (unsigned 16bit integer=w385:u16)
            }
          }
          frame #2 {
            w443 = 4 ("length")
            w442 = 8 ("length")
            n250 = Multiply(x=w438, y="ISO") -> (x*y=w437:dbl[])
            n251 = To Unsigned Word Integer(number=w437) -> (unsigned 16bit integer=w436:u16[])
            n252 = for {
              N: 110 -> [_]
              tunnel: [w465] -> w423 mode=indexing
              shift-right: [w464] -> _
              shift-left: w436 -> [w468]
              n253 = Delete From Array(array=w468, length=880, index=0) -> (deleted portion=w465:u16[], array with subset deleted=w464:u16[])
            }
            "FRAME" <- w423
            n254 = for {
              tunnel: w423 -> [w460] mode=indexing
              tunnel: [w459] -> w448 mode=indexing
              n255 = for {
                N: 880 -> [_]
                tunnel: [w463] -> w459 mode=indexing
                tunnel: w460 -> [w462] mode=indexing
                n256 = Bundle(w462, w462, w462, w462) -> (w463:cluster{u16, u16, u16, u16})  [unwired: 1 in]
              }
            }
            "OUT" <- w448
            n257 = Multiply(x=w442, y=w443) -> (x*y=w427:i32)
            n258 = Array Subset(array=w423, index (row)=101 ("index"), length (row)=w442, index (col)=9 ("index"), length (col)=w443) -> (w445:u16[][])
            n259 = Array Subset(array=w423, index (row)=101 ("index"), length (row)=8 ("length"), index (col)=9 ("index"), length (col)=4 ("length")) -> (w434:u16[][])
            n260 = Reshape Array(w445, w427) -> (w446:u16[])
            n261 = Reshape Array(w434, w427) -> (w430:u16[])
            n262 = for {
              tunnel: w446 -> [w458] mode=indexing
              shift-right: [w456] -> w447
              shift-left: u64 0 -> [w457]
              n263 = Add(x=w458, y=w457) -> (x+y=w456:u64)
            }
            n264 = Divide(x=w447, y=w427) -> (x/y=w424:dbl)
            "Среднее" <- w424
            n265 = for {
              tunnel: w424 -> [w454]
              tunnel: w430 -> [w455] mode=indexing
              shift-right: [w450] -> w435
              shift-left: 0.0 -> [w452]
              n266 = Subtract(x=w455, y=w454) -> (x-y=w453:dbl)
              n267 = Square(x=w453) -> (x^2=w451:dbl)
              n268 = Add(x=w451, y=w452) -> (x+y=w450:dbl)
            }
            n269 = Divide(x=w435, y=w427) -> (x/y=w426:dbl)
            n270 = Square Root(x=w426) -> (sqrt(x)=→"СКО":dbl)
          }
          frame #3 {
            w471 = T5 6 items=["Grayscale (U8)", "Grayscale (I16)", "Grayscale (SGL)", "Complex (CSG)", "RGB (U32)", "HSL (U32)", "RGB (U64)"] ("Image Type")
            n271 = call "IMAQ Create"("Image Name"="FPZC", "Image Type"=w471) -> ("New Image"=w473:T1)  [unwired: 3 in, 1 out]
            n272 = call "IMAQ ArrayToColorImage"("Image"=w473, "Image Pixels (U64)"=w470) -> ("Image Out"=w469:T1)  [unwired: 3 in, 1 out]
            "Image" <- w469
          }
          frame #4 {
            n273 = case shown="True" "Запись Кадра" {
              tunnel: w474 -> [_ w479]
              frame False {
              }
              frame True {
                w484 = i16 0 ("precision (6)")
                w478 = "_"
                n274 = local read "Между кадрами, мс"() -> (w496:u8)
                n275 = local read "Номер образца"() -> (w490:string)
                n276 = Concatenate Strings("Образец_" ("string"), w490) -> (w485:string)
                n277 = Get Date/Time In Seconds() -> (seconds since 1Jan1904=w493:timestamp)
                n278 = Build Path(base path="Frames", name or relative path=w485) -> (appended path=w489:path)
                n279 = Number To Fractional String(number=w496, width (-)=w484, precision (6)=w484) -> (F-format string=w497:string)  [unwired: 1 in]
                n280 = Format Date/Time String(time format string (%c)="%H.%M.%S", seconds (now)=w493) -> (date/time string=w495:string)  [unwired: 1 in]
                n281 = call <vilib>:"Check if File or Folder Exists.vi"("path"=w489) -> ("file or folder exists?"=w488:bool, "dup path"=w487:path)  [unwired: 8 in, 1 out]
                n282 = case shown="False" w488 {
                  tunnel: w487 -> [w500 w501]
                  tunnel: [w499 w501] -> w494
                  frame False {
                    n283 = Create Folder(path (use dialog)=w500) -> (created path=w499:path)  [unwired: 2 in, 2 out]
                  }
                  frame True {
                  }
                }
                n284 = Concatenate Strings(w495, w478, "Тн=" ("string"), w497, "мс_" ("string"), "ПРИМЕЧАНИЕ", w478, "Какая фотка?", ".tiff" ("element")) -> (w491:string)
                n285 = Build Path(base path=w494, name or relative path=w491) -> (appended path=w492:path)
                n286 = call-poly "IMAQ Write File 2"("File Path"=w492, "Image"=w479) -> ()  [unwired: 8 in, 2 out]
              }
            }
          }
          frame #5 {
            "FRAME_OK" <- TRUE
          }
        }
      }
    }
    n287 = local read "Стоп"() -> (w367:bool)
  }
  n288 = while {
    tunnel: w9 -> [w509]
    shift-right: ["Прошить АЦП"] -> _
    shift-left: FALSE -> [w508]
    tunnel: [w503] -> w4
    tunnel: w5 -> [_]
    stop <- w510 stop-if-true
    n289 = Greater?(x="Прошить АЦП", y=w508) -> (0:w506:bool)
    n290 = local read "Питание"() -> (w504:bool)
    n291 = And(x=w504, y=w506) -> (x .and. y?=w505:bool)
    n292 = case shown="True" w505 {
      tunnel: w509 -> [w511 w514]
      tunnel: [w511 w513] -> w503
      frame False {
        n293 = Wait (ms)(milliseconds to wait=u32 1) -> ()  [unwired: 1 out]
      }
      frame True {
        n294 = stacked-sequence {
          tunnel: w514 -> [w540 w580 w594 w623 w667 w677 w702 w736 _]
          tunnel: [_ _ _ _ _ _ _ w727 _] -> w513
          frame #0 {
            w536 = TRUE ("element")
            w537 = FALSE
            # "8"
            # "0"
            # "Configuration"
            n295 = xnode "Read/Write Control"("FPGA VI Reference In"=w540, "Enum"=T6."Configuration") -> ("FPGA VI Reference Out"=w527:refnum<k20>)  [unwired: 1 in, 1 out]
            n296 = xnode "Read/Write Control"("FPGA VI Reference In"=w517, "Read(T)/Write(F)"=TRUE) -> ("FPGA VI Reference Out"=w523:refnum<k20>, "error out"=w522:errorcluster)  [unwired: 1 in]
            n297 = case shown="\"3CH\", Default" "3CH/1CH" {
              tunnel: [TRUE FALSE] -> w535
              frame "3CH", Default {
              }
              frame "1CH" {
              }
            }
            n298 = case shown="\"4V\"" "2/4 V" {
              tunnel: [FALSE TRUE] -> w533
              frame "2V", Default {
              }
              frame "4V" {
              }
            }
            n299 = xnode "Read/Write Control"("FPGA VI Reference In"=w527, "Read(T)/Write(F)"=FALSE) -> ("FPGA VI Reference Out"=w525:refnum<k20>)  [unwired: 1 in, 1 out]
            n300 = flat-sequence {
              tunnel: w523 -> [w552]
              tunnel: w522 -> [w551]
              tunnel: [w550] -> w521
              tunnel: [w549] -> w520
              frame #0 {
                n301 = xnode "Read/Write Control"("FPGA VI Reference In"=w552, "error in"=w551, "Конфигурация"=TRUE) -> ("FPGA VI Reference Out"=w550:refnum<k20>, "error out"=w549:errorcluster)
                n302 = Wait (ms)(milliseconds to wait=u32 10) -> ()  [unwired: 1 out]
              }
            }
            n303 = Build Array(w537, w537, w537, w536, w536, w535, w536, w533, FALSE) -> (w538:bool[])
            n304 = Reverse 1D Array(array=w538) -> (reversed array=w530:bool[])
            n305 = xnode "Read/Write Control"("FPGA VI Reference In"=w525, "Write Data"=w530) -> ("FPGA VI Reference Out"=w529:refnum<k20>)  [unwired: 1 in, 1 out]
            n306 = flat-sequence {
              tunnel: w521 -> [w546]
              tunnel: w520 -> [w545]
              tunnel: [w543] -> w519
              tunnel: [w542] -> w518
              frame #0 {
                n307 = xnode "Read/Write Control"("FPGA VI Reference In"=w546, "error in"=w545, "Конфигурация"=FALSE) -> ("FPGA VI Reference Out"=w543:refnum<k20>, "error out"=w542:errorcluster)
                n308 = Wait (ms)(milliseconds to wait=u32 10) -> ()  [unwired: 1 out]
              }
            }
            n309 = flat-sequence {
              tunnel: w529 -> [w560]
              tunnel: [w558] -> w528
              frame #0 {
                n310 = xnode "Read/Write Control"("FPGA VI Reference In"=w560, "Конфигурация"=TRUE) -> ("FPGA VI Reference Out"=w558:refnum<k20>)  [unwired: 1 in, 1 out]
                n311 = Wait (ms)(milliseconds to wait=u32 10) -> ()  [unwired: 1 out]
              }
            }
            n312 = local write "АЦП прошит!"(FALSE ("АЦП прошит!")) -> ()
            n313 = xnode "Read/Write Control"("FPGA VI Reference In"=w519, "error in"=w518) -> ("READ"=→"Configuration":bool[])  [unwired: 2 out]
            n314 = flat-sequence {
              tunnel: w528 -> [w556]
              tunnel: [w554] -> w517
              frame #0 {
                n315 = xnode "Read/Write Control"("FPGA VI Reference In"=w556, "Конфигурация"=FALSE) -> ("FPGA VI Reference Out"=w554:refnum<k20>)  [unwired: 1 in, 1 out]
                n316 = Wait (ms)(milliseconds to wait=u32 10) -> ()  [unwired: 1 out]
              }
            }
          }
          frame #1 {
            # "GREEN_OFFSET"
            n317 = case shown="\"-\", Default" "+/- OUT2" {
              tunnel: [TRUE FALSE] -> w567
              frame "-", Default {
              }
              frame "+" {
              }
            }
            n318 = Quotient & Remainder(x="Смещение, до 300_OUT2", y=1.171875) -> (floor(x/y)=w572:dbl)  [unwired: 1 out]
            n319 = xnode "Read/Write Control"("FPGA VI Reference In"=w580, "Enum"=T6."GREEN OFF" ("OFFSET")) -> ("FPGA VI Reference Out"=w579:refnum<k20>, "error out"=w578:errorcluster)  [unwired: 1 in]
            n320 = Subtract(x=w572, y=1.0) -> (x-y=w569:dbl)
            n321 = To Unsigned Byte Integer(number=w569) -> (unsigned 8bit integer=w568:u8)
            n322 = xnode "Read/Write Control"("FPGA VI Reference In"=w579, "error in"=w578, "Read(T)/Write(F)"=FALSE) -> ("FPGA VI Reference Out"=w577:refnum<k20>)  [unwired: 1 out]
            n323 = Number To Boolean Array(number=w568) -> (Boolean array=w566:bool[])
            n324 = Reverse 1D Array(array=w566) -> (reversed array=w565:bool[])
            n325 = Build Array (concatenate)(w567, w565) -> (w570:bool[])
            n326 = xnode "Read/Write Control"("FPGA VI Reference In"=w577, "Write Data"=w570) -> ("FPGA VI Reference Out"=w582:refnum<k20>)  [unwired: 1 in, 1 out]
            n327 = flat-sequence {
              tunnel: w582 -> [w593]
              tunnel: [w591] -> w581
              frame #0 {
                n328 = xnode "Read/Write Control"("FPGA VI Reference In"=w593, "Конфигурация"=TRUE) -> ("FPGA VI Reference Out"=w591:refnum<k20>)  [unwired: 1 in, 1 out]
                n329 = Wait (ms)(milliseconds to wait=u32 10) -> ()  [unwired: 1 out]
              }
            }
            n330 = flat-sequence {
              tunnel: w581 -> [w589]
              tunnel: [w587] -> _
              frame #0 {
                n331 = xnode "Read/Write Control"("FPGA VI Reference In"=w589, "Конфигурация"=FALSE) -> ("FPGA VI Reference Out"=w587:refnum<k20>)  [unwired: 1 in, 1 out]
                n332 = Wait (ms)(milliseconds to wait=u32 10) -> ()  [unwired: 1 out]
              }
            }
          }
          frame #2 {
            # "RED_OFFSET"
            n333 = case shown="\"-\", Default" "+/- OUT3" {
              tunnel: [TRUE FALSE] -> w610
              frame "-", Default {
              }
              frame "+" {
              }
            }
            n334 = Quotient & Remainder(x="Смещение, до 300_OUT3", y=1.171875) -> (floor(x/y)=w605:dbl)  [unwired: 1 out]
            n335 = xnode "Read/Write Control"("FPGA VI Reference In"=w594, "Enum"=T6."RED OFF" ("OFFSET")) -> ("FPGA VI Reference Out"=w601:refnum<k20>, "error out"=w602:errorcluster)  [unwired: 1 in]
            n336 = Subtract(x=w605, y=1.0) -> (x-y=w608:dbl)
            n337 = To Unsigned Byte Integer(number=w608) -> (unsigned 8bit integer=w609:u8)
            n338 = xnode "Read/Write Control"("FPGA VI Reference In"=w601, "error in"=w602, "Read(T)/Write(F)"=FALSE) -> ("FPGA VI Reference Out"=w603:refnum<k20>)  [unwired: 1 out]
            n339 = Number To Boolean Array(number=w609) -> (Boolean array=w611:bool[])
            n340 = Reverse 1D Array(array=w611) -> (reversed array=w612:bool[])
            n341 = Build Array (concatenate)(w610, w612) -> (w607:bool[])
            n342 = xnode "Read/Write Control"("FPGA VI Reference In"=w603, "Write Data"=w607) -> ("FPGA VI Reference Out"=w599:refnum<k20>)  [unwired: 1 in, 1 out]
            n343 = flat-sequence {
              tunnel: w599 -> [w622]
              tunnel: [w620] -> w600
              frame #0 {
                n344 = xnode "Read/Write Control"("FPGA VI Reference In"=w622, "Конфигурация"=TRUE) -> ("FPGA VI Reference Out"=w620:refnum<k20>)  [unwired: 1 in, 1 out]
                n345 = Wait (ms)(milliseconds to wait=u32 10) -> ()  [unwired: 1 out]
              }
            }
            n346 = flat-sequence {
              tunnel: w600 -> [w618]
              tunnel: [w616] -> _
              frame #0 {
                n347 = xnode "Read/Write Control"("FPGA VI Reference In"=w618, "Конфигурация"=FALSE) -> ("FPGA VI Reference Out"=w616:refnum<k20>)  [unwired: 1 in, 1 out]
                n348 = Wait (ms)(milliseconds to wait=u32 10) -> ()  [unwired: 1 out]
              }
            }
          }
          frame #3 {
            # "BLUE_OFFSET"
            n349 = case shown="\"-\", Default" "+/- OUT1" {
              tunnel: [TRUE FALSE] -> w639
              frame "-", Default {
              }
              frame "+" {
              }
            }
            n350 = Quotient & Remainder(x="Смещение, до 300_OUT1", y=1.171875) -> (floor(x/y)=w634:dbl)  [unwired: 1 out]
            n351 = xnode "Read/Write Control"("FPGA VI Reference In"=w623, "Enum"=T6."BLUE OFF" ("OFFSET")) -> ("FPGA VI Reference Out"=w630:refnum<k20>, "error out"=w631:errorcluster)  [unwired: 1 in]
            n352 = Subtract(x=w634, y=1.0) -> (x-y=w637:dbl)
            n353 = To Unsigned Byte Integer(number=w637) -> (unsigned 8bit integer=w638:u8)
            n354 = xnode "Read/Write Control"("FPGA VI Reference In"=w630, "error in"=w631, "Read(T)/Write(F)"=FALSE) -> ("FPGA VI Reference Out"=w632:refnum<k20>)  [unwired: 1 out]
            n355 = Number To Boolean Array(number=w638) -> (Boolean array=w640:bool[])
            n356 = Reverse 1D Array(array=w640) -> (reversed array=w641:bool[])
            n357 = Build Array (concatenate)(w639, w641) -> (w636:bool[])
            n358 = xnode "Read/Write Control"("FPGA VI Reference In"=w632, "Write Data"=w636) -> ("FPGA VI Reference Out"=w628:refnum<k20>)  [unwired: 1 in, 1 out]
            n359 = flat-sequence {
              tunnel: w628 -> [w651]
              tunnel: [w649] -> w629
              frame #0 {
                n360 = xnode "Read/Write Control"("FPGA VI Reference In"=w651, "Конфигурация"=TRUE) -> ("FPGA VI Reference Out"=w649:refnum<k20>)  [unwired: 1 in, 1 out]
                n361 = Wait (ms)(milliseconds to wait=u32 10) -> ()  [unwired: 1 out]
              }
            }
            n362 = flat-sequence {
              tunnel: w629 -> [w647]
              tunnel: [w645] -> _
              frame #0 {
                n363 = xnode "Read/Write Control"("FPGA VI Reference In"=w647, "Конфигурация"=FALSE) -> ("FPGA VI Reference Out"=w645:refnum<k20>)  [unwired: 1 in, 1 out]
                n364 = Wait (ms)(milliseconds to wait=u32 10) -> ()  [unwired: 1 out]
              }
            }
          }
          frame #4 {
            w662 = FALSE
            # "GREEN PGA"
            n365 = Decrement(x="Усиление (до 6)_OUT2") -> (x-1=w654:u8)
            n366 = Multiply(x=w654, y=378) -> (x*y=w656:i32)
            n367 = Multiply(x="Усиление (до 6)_OUT2", y=5) -> (x*y=w659:i32)
            n368 = xnode "Read/Write Control"("FPGA VI Reference In"=w667, "Enum"=T6."GREEN PGA" ("PGA")) -> ("FPGA VI Reference Out"=w665:refnum<k20>)  [unwired: 1 in, 1 out]
            n369 = Divide(x=w656, y=w659) -> (x/y=w660:dbl)
            n370 = Number To Boolean Array(number=w660) -> (Boolean array=w653:bool[])
            n371 = xnode "Read/Write Control"("FPGA VI Reference In"=w665, "Read(T)/Write(F)"=FALSE) -> ("FPGA VI Reference Out"=w664:refnum<k20>)  [unwired: 1 in, 1 out]
            n372 = Build Array (concatenate)(w662, w662, w662, w653) -> (w661:bool[])
            n373 = xnode "Read/Write Control"("FPGA VI Reference In"=w664, "Write Data"=w661) -> ("FPGA VI Reference Out"=w666:refnum<k20>)  [unwired: 1 in, 1 out]
            n374 = flat-sequence {
              tunnel: [w675] -> w668
              tunnel: w666 -> [w674]
              frame #0 {
                n375 = xnode "Read/Write Control"("FPGA VI Reference In"=w674, "Конфигурация"=TRUE) -> ("FPGA VI Reference Out"=w675:refnum<k20>)  [unwired: 1 in, 1 out]
                n376 = Wait (ms)(milliseconds to wait=u32 10) -> ()  [unwired: 1 out]
              }
            }
            n377 = flat-sequence {
              tunnel: w668 -> [w672]
              tunnel: [w670] -> _
              frame #0 {
                n378 = xnode "Read/Write Control"("FPGA VI Reference In"=w672, "Конфигурация"=FALSE) -> ("FPGA VI Reference Out"=w670:refnum<k20>)  [unwired: 1 in, 1 out]
                n379 = Wait (ms)(milliseconds to wait=u32 10) -> ()  [unwired: 1 out]
              }
            }
          }
          frame #5 {
            w680 = FALSE
            # "BLUE PGA"
            n380 = Decrement(x="Усиление (до 6)_OUT1") -> (x-1=w684:u8)
            n381 = Multiply(x=w684, y=378) -> (x*y=w685:i32)
            n382 = Multiply(x="Усиление (до 6)_OUT1", y=5) -> (x*y=w687:i32)
            n383 = xnode "Read/Write Control"("FPGA VI Reference In"=w677, "Enum"=T6."BLUE PGA" ("PGA")) -> ("FPGA VI Reference Out"=w691:refnum<k20>)  [unwired: 1 in, 1 out]
            n384 = Divide(x=w685, y=w687) -> (x/y=w688:dbl)
            n385 = Number To Boolean Array(number=w688) -> (Boolean array=w683:bool[])
            n386 = xnode "Read/Write Control"("FPGA VI Reference In"=w691, "Read(T)/Write(F)"=FALSE) -> ("FPGA VI Reference Out"=w690:refnum<k20>)  [unwired: 1 in, 1 out]
            n387 = Build Array (concatenate)(w680, w680, w680, w683) -> (w689:bool[])
            n388 = xnode "Read/Write Control"("FPGA VI Reference In"=w690, "Write Data"=w689) -> ("FPGA VI Reference Out"=w692:refnum<k20>)  [unwired: 1 in, 1 out]
            n389 = flat-sequence {
              tunnel: [w700] -> w693
              tunnel: w692 -> [w699]
              frame #0 {
                n390 = xnode "Read/Write Control"("FPGA VI Reference In"=w699, "Конфигурация"=TRUE) -> ("FPGA VI Reference Out"=w700:refnum<k20>)  [unwired: 1 in, 1 out]
                n391 = Wait (ms)(milliseconds to wait=u32 10) -> ()  [unwired: 1 out]
              }
            }
            n392 = flat-sequence {
              tunnel: w693 -> [w697]
              tunnel: [w695] -> _
              frame #0 {
                n393 = xnode "Read/Write Control"("FPGA VI Reference In"=w697, "Конфигурация"=FALSE) -> ("FPGA VI Reference Out"=w695:refnum<k20>)  [unwired: 1 in, 1 out]
                n394 = Wait (ms)(milliseconds to wait=u32 10) -> ()  [unwired: 1 out]
              }
            }
          }
          frame #6 {
            w713 = FALSE
            # "RED PGA"
            n395 = Decrement(x="Усиление (до 6)_OUT3") -> (x-1=w705:u8)
            n396 = Multiply(x=w705, y=378) -> (x*y=w707:i32)
            n397 = Multiply(x="Усиление (до 6)_OUT3", y=5) -> (x*y=w710:i32)
            n398 = xnode "Read/Write Control"("FPGA VI Reference In"=w702, "Enum"=T6."RED PGA" ("PGA")) -> ("FPGA VI Reference Out"=w716:refnum<k20>)  [unwired: 1 in, 1 out]
            n399 = Divide(x=w707, y=w710) -> (x/y=w711:dbl)
            n400 = Number To Boolean Array(number=w711) -> (Boolean array=w704:bool[])
            n401 = xnode "Read/Write Control"("FPGA VI Reference In"=w716, "Read(T)/Write(F)"=FALSE) -> ("FPGA VI Reference Out"=w715:refnum<k20>)  [unwired: 1 in, 1 out]
            n402 = Build Array (concatenate)(w713, w713, w713, w704) -> (w712:bool[])
            n403 = xnode "Read/Write Control"("FPGA VI Reference In"=w715, "Write Data"=w712) -> ("FPGA VI Reference Out"=w717:refnum<k20>)  [unwired: 1 in, 1 out]
            n404 = flat-sequence {
              tunnel: [w725] -> w718
              tunnel: w717 -> [w724]
              frame #0 {
                n405 = xnode "Read/Write Control"("FPGA VI Reference In"=w724, "Конфигурация"=TRUE) -> ("FPGA VI Reference Out"=w725:refnum<k20>)  [unwired: 1 in, 1 out]
                n406 = Wait (ms)(milliseconds to wait=u32 10) -> ()  [unwired: 1 out]
              }
            }
            n407 = flat-sequence {
              tunnel: w718 -> [w722]
              tunnel: [w720] -> _
              frame #0 {
                n408 = xnode "Read/Write Control"("FPGA VI Reference In"=w722, "Конфигурация"=FALSE) -> ("FPGA VI Reference Out"=w720:refnum<k20>)  [unwired: 1 in, 1 out]
                n409 = Wait (ms)(milliseconds to wait=u32 10) -> ()  [unwired: 1 out]
              }
            }
          }
          frame #7 {
            # "MUX"
            n410 = xnode "Read/Write Control"("FPGA VI Reference In"=w736, "Enum"=T6."MUX") -> ("FPGA VI Reference Out"=w730:refnum<k20>)  [unwired: 1 in, 1 out]
            n411 = case shown="\"OUT3\"" "Какой канал?" {
              tunnel: [bool[] [FALSE, TRUE, FALSE, FALSE, TRUE, FALSE, FALSE, FALSE, FALSE] ("MUX_register") bool[] [FALSE, TRUE, FALSE, TRUE, FALSE, FALSE, FALSE, FALSE, FALSE] ("MUX_register") bool[] [FALSE, TRUE, TRUE, FALSE, FALSE, FALSE, FALSE, FALSE, FALSE] ("MUX_register")] -> w728
              frame "OUT1", Default {
              }
              frame "OUT2" {
              }
              frame "OUT3" {
              }
            }
            n412 = xnode "Read/Write Control"("FPGA VI Reference In"=w730, "Read(T)/Write(F)"=FALSE) -> ("FPGA VI Reference Out"=w732:refnum<k20>)  [unwired: 1 in, 1 out]
            n413 = xnode "Read/Write Control"("FPGA VI Reference In"=w732, "Write Data"=w728) -> ("FPGA VI Reference Out"=w733:refnum<k20>)  [unwired: 1 in, 1 out]
            n414 = flat-sequence {
              tunnel: [w746] -> w734
              tunnel: w733 -> [w745]
              frame #0 {
                n415 = xnode "Read/Write Control"("FPGA VI Reference In"=w745, "Конфигурация"=TRUE) -> ("FPGA VI Reference Out"=w746:refnum<k20>)  [unwired: 1 in, 1 out]
                n416 = Wait (ms)(milliseconds to wait=u32 10) -> ()  [unwired: 1 out]
              }
            }
            n417 = flat-sequence {
              tunnel: w734 -> [w743]
              tunnel: [w741] -> w727
              frame #0 {
                n418 = xnode "Read/Write Control"("FPGA VI Reference In"=w743, "Конфигурация"=FALSE) -> ("FPGA VI Reference Out"=w741:refnum<k20>)  [unwired: 1 in, 1 out]
                n419 = Wait (ms)(milliseconds to wait=u32 10) -> ()  [unwired: 1 out]
              }
            }
          }
          frame #8 {
            "АЦП прошит!" <- TRUE ("АЦП прошит!")
          }
        }
      }
    }
    n420 = local read "Стоп"() -> (w510:bool)
  }
  n421 = while {
    tunnel: w9 -> [w752]
    shift-right: [w750] -> _
    shift-left: enum16{"1", "2", "3", "4"}."1" -> [w751]
    tunnel: [w749] -> w1
    tunnel: w5 -> [_]
    stop <- w754 stop-if-true
    n422 = case shown="True" "ПЕРЕБОР?" {
      tunnel: w752 -> [w755 w767]
      tunnel: w751 -> [w756 w766]
      tunnel: [w756 w762] -> w750
      tunnel: [w755 w761] -> w749
      frame False {
        n423 = Wait (ms)(milliseconds to wait=u32 50) -> ()  [unwired: 1 out]
      }
      frame True {
        n424 = flat-sequence {
          tunnel: w767 -> [w770]
          tunnel: w766 -> [w774]
          tunnel: [w773] -> w765
          tunnel: [w768] -> w758
          tunnel: w765 -> [w792]
          tunnel: [w792] -> w763
          tunnel: [w791] -> w759
          tunnel: w758 -> [w791]
          tunnel: [w795] -> w764
          tunnel: w763 -> [w795]
          tunnel: [w794] -> w760
          tunnel: w759 -> [w794]
          tunnel: w764 -> [w799]
          tunnel: [w799] -> w762
          tunnel: [w798] -> w761
          tunnel: w760 -> [w798]
          frame #0 {
            n425 = case shown="\"4\"" w774 {
              tunnel: [enum16{"1", "2", "3", "4"}."2" enum16{"1", "2", "3", "4"}."3" enum16{"1", "2", "3", "4"}."4" enum16{"1", "2", "3", "4"}."1"] -> w773
              tunnel: [FALSE ("VNR") FALSE ("VNR") FALSE ("VNR") TRUE ("VNR")] -> w772
              tunnel: ["1" "2" "3" "4"] -> w771
              tunnel: [enum16{"OUT1", "OUT2", "OUT3"}."OUT1" ("Какой канал?") enum16{"OUT1", "OUT2", "OUT3"}."OUT2" ("Какой канал?") enum16{"OUT1", "OUT2", "OUT3"}."OUT3" ("Какой канал?") enum16{"OUT1", "OUT2", "OUT3"}."OUT3" ("Какой канал?")] -> w769
              frame "1", Default {
              }
              frame "2" {
              }
              frame "3" {
              }
              frame "4" {
              }
            }
            "Канал" <- w771
            n426 = local write "Какой канал?"(w769) -> ()
            n427 = xnode "Read/Write Control"("FPGA VI Reference In"=w770, "VINR"=w772) -> ("FPGA VI Reference Out"=w768:refnum<k20>)  [unwired: 1 in, 1 out]
          }
          frame #1 {
            n428 = local write "Прошить АЦП"(TRUE ("Прошить АЦП")) -> ()
          }
          frame #2 {
            n429 = while {
              stop <- w797 stop-if-true
              n430 = local read "АЦП прошит!"() -> (w797:bool)
              n431 = Wait (ms)(milliseconds to wait=u32 10) -> ()  [unwired: 1 out]
            }
          }
          frame #3 {
            n432 = local write "Прошить АЦП"(FALSE ("Прошить АЦП")) -> ()
            n433 = Wait (ms)(milliseconds to wait=u32 3000) -> ()  [unwired: 1 out]
          }
        }
      }
    }
    n434 = local read "Стоп"() -> (w754:bool)
  }
  n435 = while {
    tunnel: w9 -> [w835]
    tunnel: [w834] -> w3
    tunnel: w5 -> [_]
    stop <- w833 stop-if-true
    # "Общие настройки"
    n436 = local read "Питание"() -> (w837:bool)
    n437 = And(x="Линейки", y=w837) -> (x .and. y?=w831:bool)
    n438 = local read "Стоп"() -> (w832:bool)
    n439 = xnode "Read/Write Control"("FPGA VI Reference In"=w835, "Остановка основного цикла"=w832, "Линейки"=w831, "Сколько строк?"="Сколько строк?", "2017"="2017", "PS1_2"="PS1_2", "PS1_1"="PS1_1", "PS2_1"="PS2_1", "PS2_2"="PS2_2", "PS3_1"="PS3_1", "PS3_2"="PS3_2", "PS4_1"="PS4_1", "PS4_2"="PS4_2", "CDS1_2"="CDS1_2", "CDS1_1"="CDS1_1", "CDS2_2"="CDS2_2", "CDS2_1"="CDS2_1", "ADC_2"="ADC_2", "ADC_1"="ADC_1", "RG_2"="RG_2", "RG_1"="RG_1", "PH21_2"="PH21_2", "PH21_1"="PH21_1", "PH11_2"="PH11_2", "PH11_1"="PH11_1", "HOR"="HOR", "10"="10", "LOW"="LOW", "HIGH"="HIGH", "Между кадрами"="Между кадрами, мс", "LED"="LED") -> ("FPGA VI Reference Out"=w834:refnum<k20>)  [unwired: 1 in, 1 out]
    n440 = Wait (ms)(milliseconds to wait=u32 1) -> ()  [unwired: 1 out]
    n441 = local read "Стоп"() -> (w833:bool)
  }
  n442 = flat-sequence {
    tunnel: w4 -> [w838]
    tunnel: w3 -> [_]
    tunnel: w2 -> [_]
    tunnel: w1 -> [_]
    frame #0 {
      n443 = xnode "Close FPGA VI Reference"("FPGA VI Reference In"=w838) -> ()  [unwired: 1 in, 1 out]
    }
  }
  n444 = call <instrlib>:"niDCPower Close.vi"("instrument handle"=w13) -> ()  [unwired: 10 in, 1 out]
  n445 = call <instrlib>:"niDCPower Close.vi"("instrument handle"=w14) -> ()  [unwired: 10 in, 1 out]
  n446 = call <instrlib>:"niDCPower Close.vi"("instrument handle"=w15) -> ()  [unwired: 10 in, 1 out]
